vi "Refresh Statistics.vi"(11 "CIFPlugin in":refnum<class "CAN_Reader_CANsub_Plugin.lvclass">) -> (3 "CIFPlugin out":refnum<class "CAN_Reader_CANsub_Plugin.lvclass">)   [LabVIEW 2021, in "CAN_Reader_CANsub_Plugin.lvclass"]
uses:
  CAN_Reader_CANsub_Plugin.lvclass
  CAN_Reader_CANsub_Plugin.lvclass/CAN_Reader_CANsub_Plugin.ctl
  Typedef/Statistics.ctl
  <vilib>/CIF Foundation/CIF CAN RW Core/CAN_RW_CORE.lvclass
  <vilib>/CIF Foundation/CIF XNET CAN RW/XNET CAN RW.lvclass
  C:/Program Files/National Instruments/LabVIEW 2021/vi.lib/CIF Foundation/CIF CAN RW Core/CAN_RW_CORE.lvclass
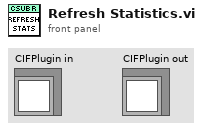
[diagram p1: front panel]
types:
  T1 = typedef "CAN_Reader_CANsub_Plugin.lvclass/Statistics.ctl" = cluster{"Iterations":u64, "Read Timeouts":u64, "Read Frames":u64, "Frames Filtered":u64}
  T2 = typedef "CAN_RW_CORE.lvclass/Statistics.ctl" = cluster{"Total Frames RW":u32, "Frames Filtered ":u32, "ACK Errors":u32}
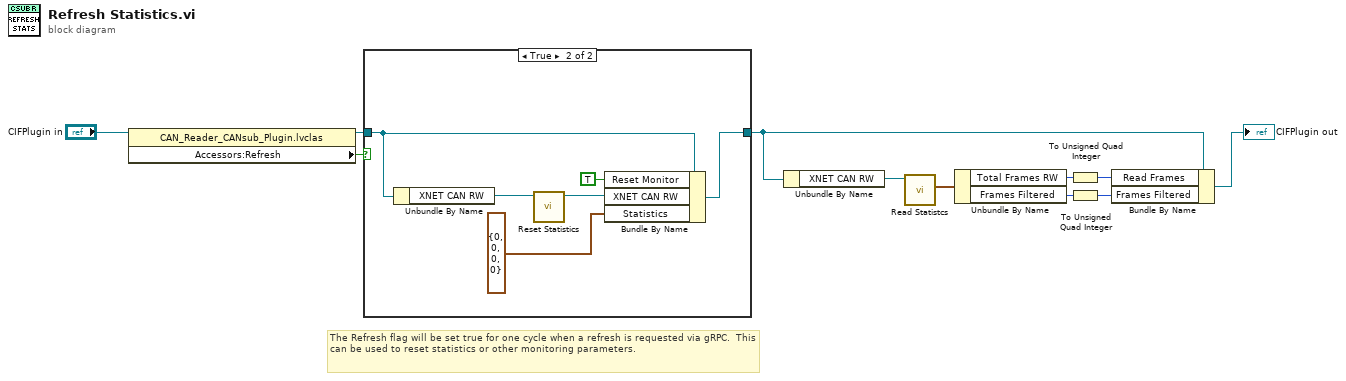
[diagram p0: block diagram]
diagram:
  # "The Refresh flag will be set true for one cycle when a refresh is requested via gRPC.  This can be used to reset statistics or other monitoring parameters."
  n1 = property class="CAN_Reader_CANsub_Plugin.lvclas"(reference="CIFPlugin in") -> (reference out=w10:refnum<class "CAN_Reader_CANsub_Plugin.lvclass">, "Accessors:Refresh"=w11:bool)  [unwired: 1 in, 1 out]
  n2 = case shown="True" w11 {
    tunnel: w10 -> [w12 w16]
    tunnel: [w12 w18] -> w5
    frame False {
    }
    frame True {
      n3 = Unbundle By Name(w16) -> ("XNET CAN RW"=w15:refnum<class "XNET CAN RW.lvclass">)
      n4 = call <vilib>:"Reset Statistics.vi"("CAN_RW_CORE in"=w15) -> ("CAN_RW_CORE out"=w14:refnum<class "XNET CAN RW.lvclass">)  [unwired: 9 in, 1 out]
      n5 = Bundle By Name(cluster=w16, "Reset Monitor"=TRUE, "XNET CAN RW"=w14, "Statistics"=T1 {"Iterations"=0, "Read Timeouts"=0, "Read Frames"=0, "Frames Filtered"=0} ("-> gRPC Comm.Cyclic Data -> gRPC .Statistics")) -> (w18:refnum<class "CAN_Reader_CANsub_Plugin.lvclass">)
    }
  }
  n6 = Unbundle By Name(w5) -> ("XNET CAN RW"=w8:refnum<class "XNET CAN RW.lvclass">)
  n7 = call <vilib>:"Read Statistcs.vi"("CAN_RW_CORE in"=w8) -> ("Statistcs"=w7:T2)  [unwired: 8 in, 2 out]
  n8 = Unbundle By Name(w7) -> ("Total Frames RW"=w6:u32, "Frames Filtered"=w2:u32)
  n9 = To Unsigned Quad Integer(1:w6) -> (0:w3:u64)
  n10 = To Unsigned Quad Integer(1:w2) -> (0:w1:u64)
  n11 = Bundle By Name(cluster=w5, "Read Frames"=w3, "Frames Filtered"=w1) -> (→"CIFPlugin out":refnum<class "CAN_Reader_CANsub_Plugin.lvclass">)
